vi "Single Axis motor_R(SubVI).vi"(0 "State=1, I":dbl, 1 "Motor=0, I":i32, 2 "Motor Input":dbl, 3 "Step diff":dbl, 4 "Motor Input_L":refnum<vi>) -> (17 "State Chart":i32(graph), 19 "right":bool, 20 "State=1, O":dbl, 21 "Motor=0, O":i32, 23 "up":bool, 24 "left":bool, 25 "Moving":bool, 26 "Motor State":dbl, 27 "down":bool)   [LabVIEW 2018]
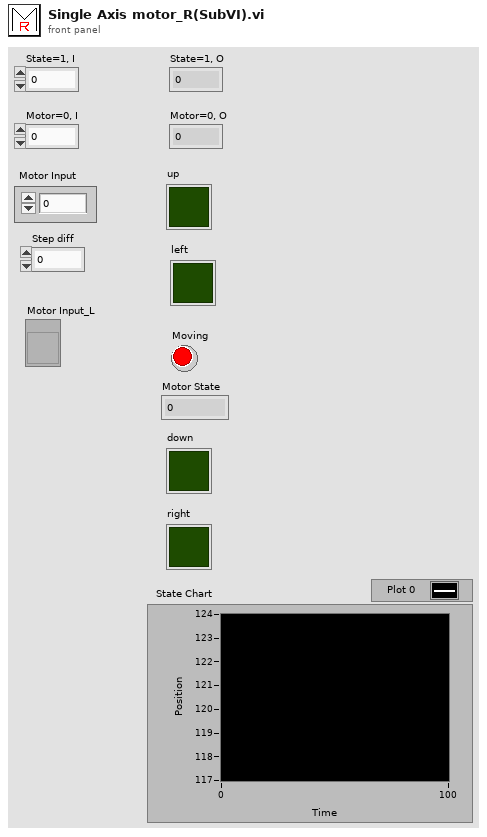
[diagram p1: front panel]
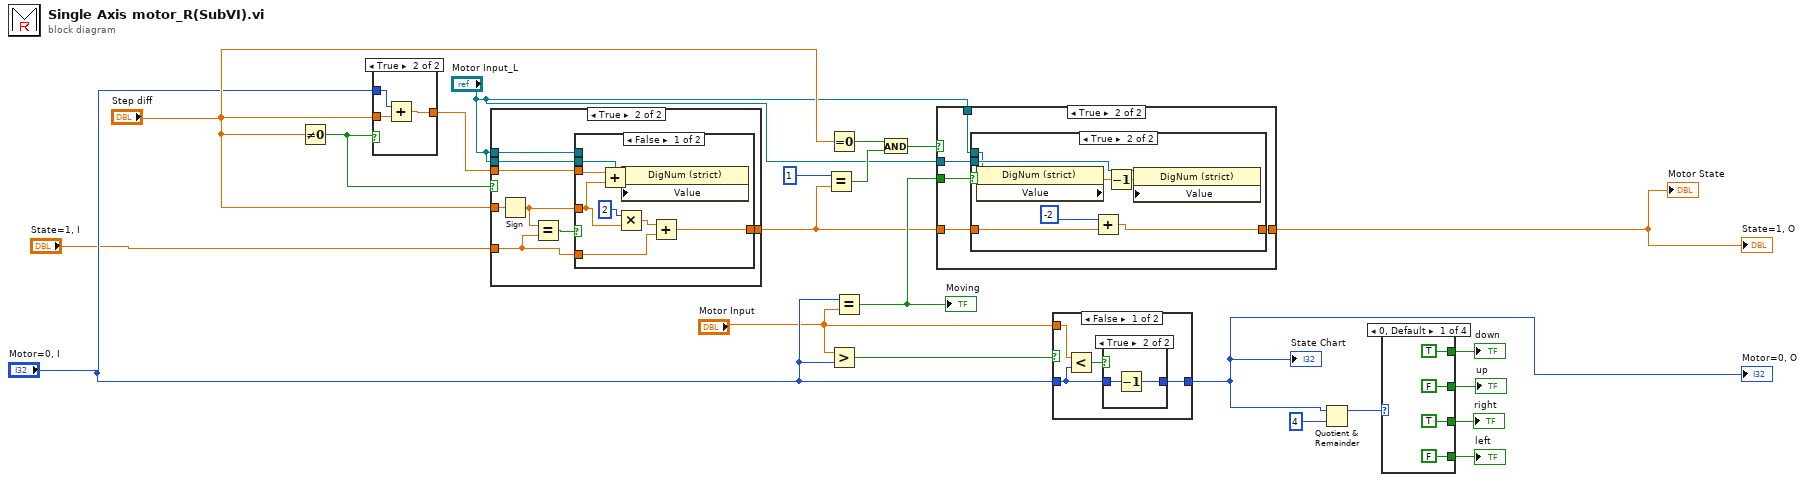
[diagram p0: block diagram]
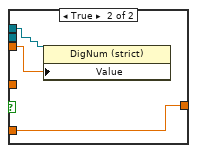
[diagram p5: hidden frame]
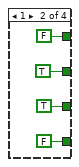
[diagram p6: hidden frame]
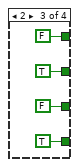
[diagram p7: hidden frame]
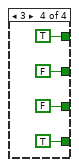
[diagram p8: hidden frame]
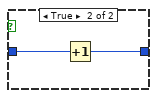
[diagram p10: hidden frame]
diagram:
  n1 = Not Equal To 0?(x="Step diff") -> (x != 0?=w4:bool)
  n2 = case shown="True" w4 {
    tunnel: "Motor=0, I" -> [_ w26]
    tunnel: "Step diff" -> [w23 w25]
    tunnel: [w23 w24] -> w5
    frame False {
    }
    frame True {
      n3 = Add(x=w26, y=w25) -> (x+y=w24:dbl)
    }
  }
  n4 = case shown="True" w4 {
    tunnel: [w27 w34] -> w12
    tunnel: "State=1, I" -> [w27 w33]
    tunnel: "Step diff" -> [_ w31]
    tunnel: w5 -> [_ w30]
    tunnel: "Motor Input_L" -> [_ w29]
    tunnel: "Motor Input_L" -> [_ w28]
    frame False {
    }
    frame True {
      n5 = Sign(1:w31) -> (0:w32:dbl)
      n6 = Equal?(x=w32, y=w33) -> (x = y?=w35:bool)
      n7 = case shown="False" w35 {
        tunnel: w32 -> [w37 _]
        tunnel: [w42 w46] -> w34
        tunnel: w33 -> [w40 w46]
        tunnel: w30 -> [w39 w45]
        tunnel: w29 -> [w36 _]
        tunnel: w28 -> [_ w44]
        frame False {
          n8 = Add(x=w39, y=w37) -> (x+y=w41:dbl)
          n9 = Multiply(x=2, y=w37) -> (x*y=w38:dbl)
          n10 = property class="DigNum (strict)"(reference=w36, "Value"=w41) -> ()  [unwired: 1 in, 2 out]
          n11 = Add(x=w38, y=w40) -> (x+y=w42:dbl)
        }
        frame True {
          n12 = property class="DigNum (strict)"(reference=w44, "Value"=w45) -> ()  [unwired: 1 in, 2 out]
        }
      }
    }
  }
  n13 = Equal?(x=1, y=w12) -> (x = y?=w11:bool)
  n14 = Equal To 0?(x="Step diff") -> (x = 0?=w10:bool)
  n15 = Greater?(x="Motor Input", y="Motor=0, I") -> (0:w3:bool)
  n16 = Equal?(x="Motor=0, I", y="Motor Input") -> (x = y?=w22:bool)
  "Moving" <- w22
  n17 = And(x=w10, y=w11) -> (x .and. y?=w9:bool)
  n18 = case shown="True" w9 {
    tunnel: w12 -> [w47 w51]
    tunnel: [w47 w52] -> w8
    tunnel: w22 -> [_ w50]
    tunnel: "Motor Input_L" -> [_ w49]
    tunnel: "Motor Input_L" -> [_ w48]
    frame False {
    }
    frame True {
      n19 = case shown="True" w50 {
        tunnel: [w53 w58] -> w52
        tunnel: w51 -> [w53 w59]
        tunnel: w49 -> [_ w55]
        tunnel: w48 -> [_ w54]
        frame False {
        }
        frame True {
          n20 = property class="DigNum (strict)"(reference=w54) -> ("Value"=w56:dbl)  [unwired: 1 in, 2 out]
          n21 = Add(x=-2, y=w59) -> (x+y=w58:dbl)
          n22 = Decrement(x=w56) -> (x-1=w57:dbl)
          n23 = property class="DigNum (strict)"(reference=w55, "Value"=w57) -> ()  [unwired: 1 in, 2 out]
        }
      }
    }
  }
  "Motor State" <- w8
  "State=1, O" <- w8
  n24 = case shown="False" w3 {
    tunnel: "Motor=0, I" -> [w62 w69]
    tunnel: [w61 w68] -> w7
    tunnel: "Motor Input" -> [w64 _]
    frame False {
      n25 = Less?(x=w64, y=w62) -> (x < y?=w63:bool)
      n26 = case shown="True" w63 {
        tunnel: w62 -> [w65 w67]
        tunnel: [w65 w66] -> w61
        frame False {
        }
        frame True {
          n27 = Decrement(x=w67) -> (x-1=w66:i32)
        }
      }
    }
    frame True {
      n28 = Increment(x=w69) -> (x+1=w68:i32)
    }
  }
  "State Chart" <- w7
  "Motor=0, O" <- w7
  n29 = Quotient & Remainder(x=w7, y=4) -> (x-y*floor(x/y)=w14:i32)  [unwired: 1 out]
  n30 = case shown="0, Default" w14 {
    tunnel: [FALSE FALSE TRUE TRUE] -> w18
    tunnel: [TRUE TRUE FALSE FALSE] -> w17
    tunnel: [FALSE TRUE TRUE FALSE] -> w16
    tunnel: [TRUE FALSE FALSE TRUE] -> w15
    frame 0, Default {
    }
    frame 1 {
    }
    frame 2 {
    }
    frame 3 {
    }
  }
  "up" <- w16
  "down" <- w15
  "right" <- w17
  "left" <- w18
